vi "Refresh Max Sizes.vi"(8 "error in (no error)":errorcluster, 11 "2DArrayManager in":refnum<class "2DArrayManager.lvclass">) -> (0 "error out":errorcluster, 3 "2DArrayManager out":refnum<class "2DArrayManager.lvclass">)   [LabVIEW 2020, in "OOPanel.lvlib" / "2DArrayManager.lvclass"]
uses:
  2DArrayManager.lvclass
  2DArrayManager.lvclass/2DArrayManager.ctl
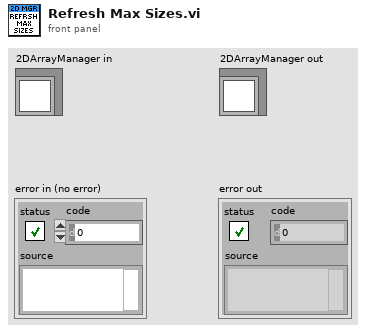
[diagram p1: front panel]
types:
  T1 = typedef "OOPanel.lvlib/Desired Size.ctl" = cluster{"Width":u32, "Height":u32}
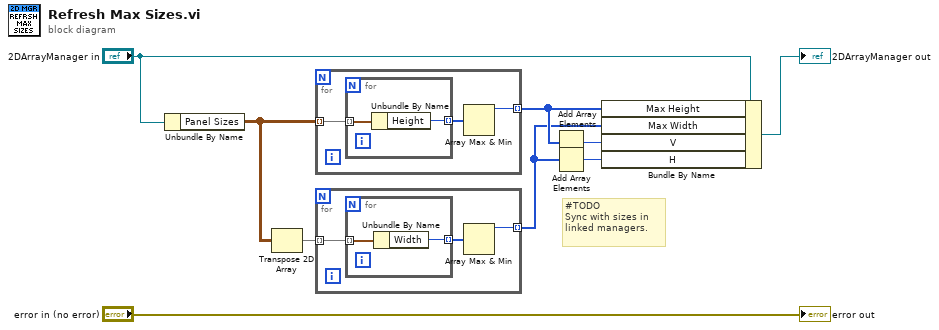
[diagram p0: block diagram]
diagram:
  # "#TODO\nSync with sizes in linked managers."
  n1 = Unbundle By Name("2DArrayManager in") -> ("Panel Sizes"=w6:T1[][])
  n2 = Transpose 2D Array(2D array=w6) -> (transposed array=w7:T1[][])
  n3 = for {
    tunnel: w6 -> [w12] mode=indexing
    tunnel: [w10] -> w4 mode=indexing
    n4 = for {
      tunnel: w12 -> [w14] mode=indexing
      tunnel: [w13] -> w11 mode=indexing
      n5 = Unbundle By Name(w14) -> ("Height"=w13:u32)
    }
    n6 = Array Max & Min(array=w11) -> (max value=w10:u32)  [unwired: 3 out]
  }
  n7 = for {
    tunnel: w7 -> [w17] mode=indexing
    tunnel: [w15] -> w3 mode=indexing
    n8 = for {
      tunnel: w17 -> [w19] mode=indexing
      tunnel: [w18] -> w16 mode=indexing
      n9 = Unbundle By Name(w19) -> ("Width"=w18:u32)
    }
    n10 = Array Max & Min(array=w16) -> (max value=w15:u32)  [unwired: 3 out]
  }
  n11 = Add Array Elements(numeric array=w4) -> (sum=w2:u32)
  n12 = Add Array Elements(numeric array=w3) -> (sum=w1:u32)
  n13 = Bundle By Name(cluster="2DArrayManager in", "Max Height"=w4, "Max Width"=w3, "V"=w2, "H"=w1) -> (→"2DArrayManager out":refnum<class "2DArrayManager.lvclass">)
  "error out" <- "error in (no error)"
